vi "test progress notifications.vi"(8 "error in (no error)":errorcluster) -> (0 "error out":errorcluster, 3 "body":string)   [LabVIEW 2020, in "MCP Server tests.lvlib"]
doc: "Progress notifications over Server-Sent Events. fake_tool_progress works through 10 steps and calls Report Progress.vi before each. A tools/call with params._meta.progressToken whose Accept header contains text/event-stream is answered as text/event-stream: ten notifications/progress events carrying the progressToken exactly as sent (a string in the legacy request, a number in the modern one) with progress 1..10 in increasing order and total 10, then the JSON-RPC result as the last data event. The same call without a progressToken is answered as plain application/json. The requests are sent with the LabVIEW HTTP Client directly."
uses:
  MCP Server tests.lvlib
  <vilib>/addons/_JKI Toolkits/Caraya/classes/Test/Test.lvclass
  <vilib>/addons/_JKI Toolkits/Caraya/classes/Assert/Assert.lvclass
panel:
  out "lookup error":errorcluster
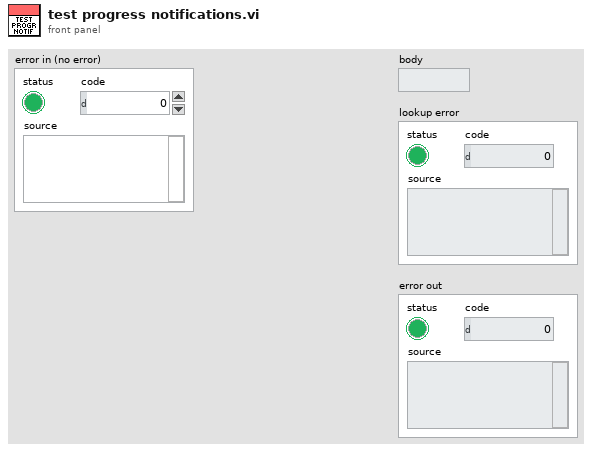
[diagram p1: front panel]
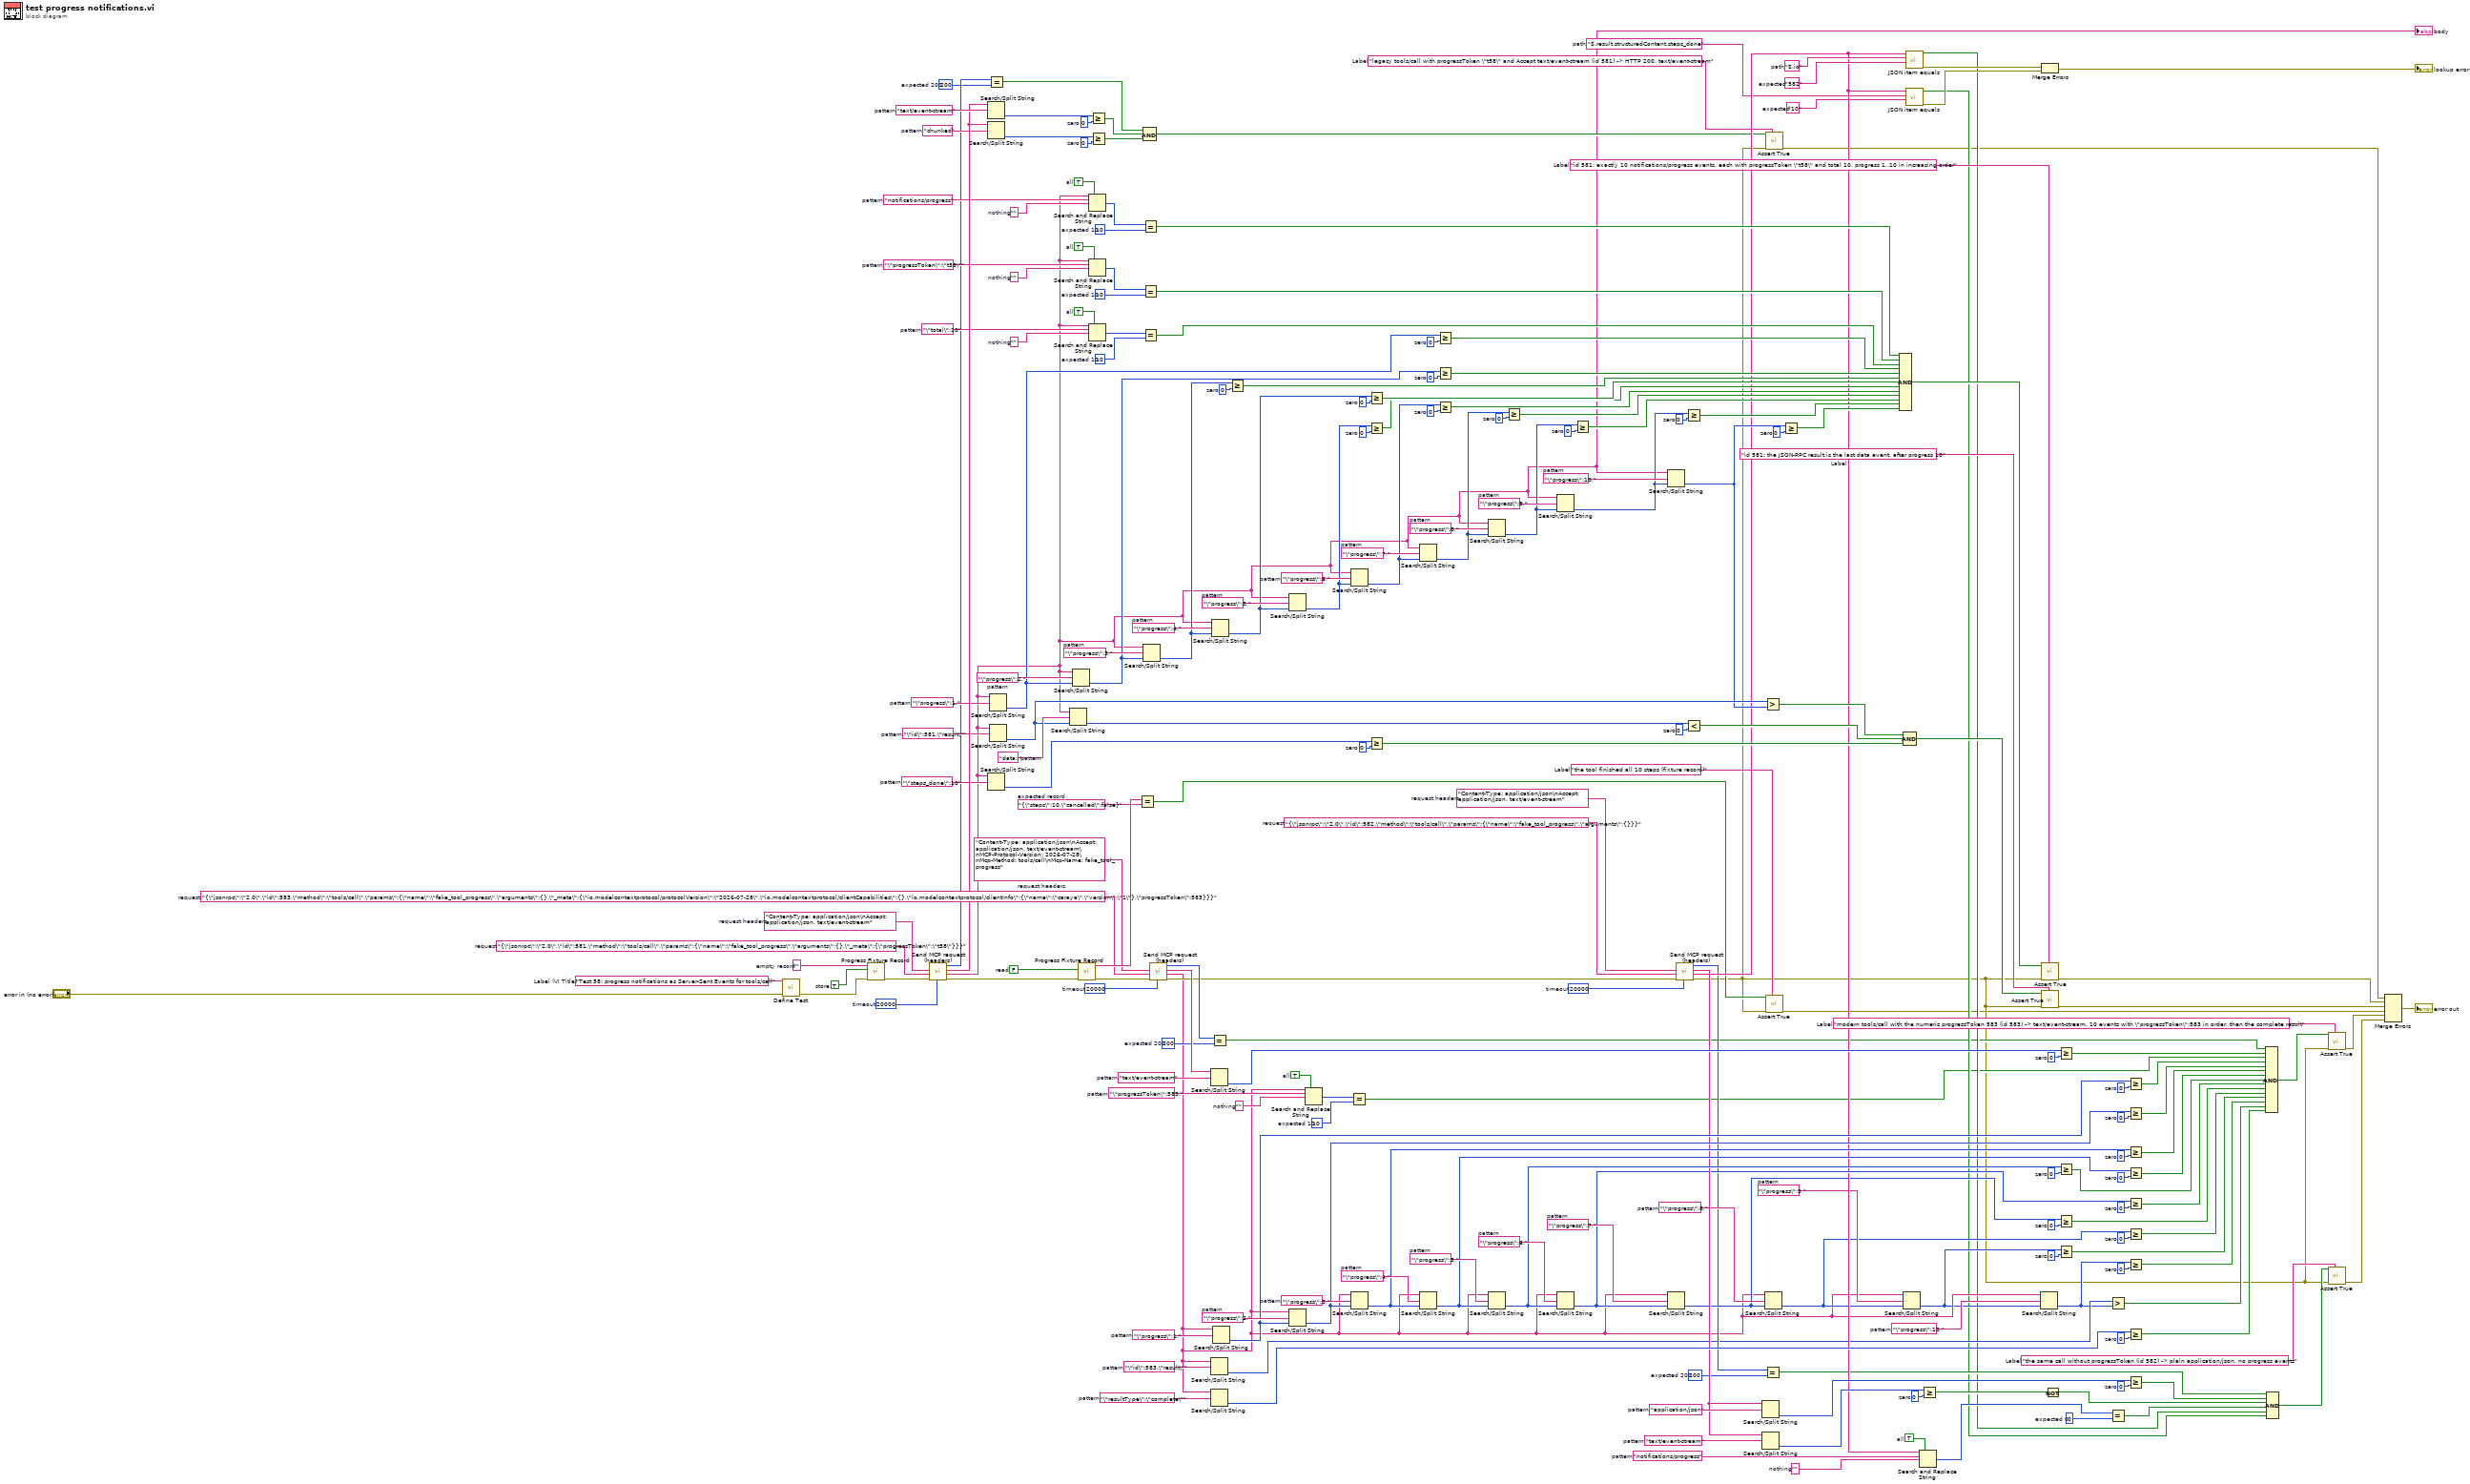
[diagram p0: block diagram]
diagram:
  w88 = "Content-Type: application/json\nAccept: application/json, text/event-stream"  # request headers
  w142 = "Content-Type: application/json\nAccept: application/json, text/event-stream\nMCP-Protocol-Version: 2026-07-28\nMcp-Method: tools/call\nMcp-Name: fake_tool_progress"  # request headers
  w209 = "Content-Type: application/json\nAccept: application/json, text/event-stream"  # request headers
  w28 = "the same call without progressToken (id 582) -> plain application/json, no progress events"  # Label
  w10 = "modern tools/call with the numeric progressToken 583 (id 583) -> text/event-stream, 10 events with \"progressToken\":583 in order, then the complete result"  # Label
  w52 = "the tool finished all 10 steps (fixture record)"  # Label
  w54 = "id 581: the JSON-RPC result is the last data event, after progress 10"  # Label
  w56 = "id 581: exactly 10 notifications/progress events, each with progressToken \"t58\" and total 10, progress 1..10 in increasing order"  # Label
  w58 = "legacy tools/call with progressToken \"t58\" and Accept text/event-stream (id 581) -> HTTP 200, text/event-stream"  # Label
  w61 = "10"  # expected
  w62 = "$.result.structuredContent.steps_done"  # path
  w65 = "582"  # expected
  w66 = "$.id"  # path
  w67 = 0  # expected 0
  w76 = TRUE  # all
  w77 = ""  # nothing
  w78 = "notifications/progress"  # pattern
  w69 = 0  # zero
  w79 = "text/event-stream"  # pattern
  w71 = 0  # zero
  w81 = "application/json"  # pattern
  w47 = 200  # expected 200
  w116 = 0  # zero
  w128 = "\"resultType\":\"complete\""  # pattern
  w129 = "\"id\":583,\"result\""  # pattern
  w118 = 10  # expected 10
  w130 = TRUE  # all
  w131 = ""  # nothing
  w132 = "\"progressToken\":583,"  # pattern
  w123 = 0  # zero
  w134 = "text/event-stream"  # pattern
  w114 = 200  # expected 200
  w38 = 0  # zero
  w40 = "\"progress\":10,"  # pattern
  w42 = 0  # zero
  w44 = "\"progress\":9,"  # pattern
  w45 = 0  # zero
  w50 = "\"progress\":8,"  # pattern
  w51 = 0  # zero
  w74 = "\"progress\":7,"  # pattern
  w75 = 0  # zero
  w83 = "\"progress\":6,"  # pattern
  w84 = 0  # zero
  w90 = "\"progress\":5,"  # pattern
  w91 = 0  # zero
  w93 = "\"progress\":4,"  # pattern
  w94 = 0  # zero
  w112 = "\"progress\":3,"  # pattern
  w113 = 0  # zero
  w121 = "\"progress\":2,"  # pattern
  w122 = 0  # zero
  w133 = "\"progress\":1,"  # pattern
  w164 = "{\"steps\":10,\"cancelled\":false}"  # expected record
  w175 = 0  # zero
  w191 = "\"steps_done\":10"  # pattern
  w166 = 0  # zero
  w183 = "data: "  # pattern
  w177 = 10  # expected 10
  w192 = TRUE  # all
  w193 = ""  # nothing
  w194 = "\"total\":10"  # pattern
  w179 = 10  # expected 10
  w195 = TRUE  # all
  w196 = ""  # nothing
  w197 = "\"progressToken\":\"t58\""  # pattern
  w181 = 10  # expected 10
  w198 = TRUE  # all
  w199 = ""  # nothing
  w200 = "notifications/progress"  # pattern
  w187 = 0  # zero
  w203 = "chunked"  # pattern
  w189 = 0  # zero
  w205 = "text/event-stream"  # pattern
  w171 = 200  # expected 200
  w201 = "\"id\":581,\"result\""  # pattern
  w127 = 0  # zero
  w137 = "\"progress\":10,"  # pattern
  w138 = 0  # zero
  w144 = "\"progress\":9,"  # pattern
  w145 = 0  # zero
  w147 = "\"progress\":8,"  # pattern
  w148 = 0  # zero
  w150 = "\"progress\":7,"  # pattern
  w151 = 0  # zero
  w153 = "\"progress\":6,"  # pattern
  w154 = 0  # zero
  w156 = "\"progress\":5,"  # pattern
  w157 = 0  # zero
  w162 = "\"progress\":4,"  # pattern
  w163 = 0  # zero
  w169 = "\"progress\":3,"  # pattern
  w170 = 0  # zero
  w185 = "\"progress\":2,"  # pattern
  w186 = 0  # zero
  w202 = "\"progress\":1,"  # pattern
  w86 = 20000  # timeout
  w87 = "{\"jsonrpc\":\"2.0\",\"id\":582,\"method\":\"tools/call\",\"params\":{\"name\":\"fake_tool_progress\",\"arguments\":{}}}"  # request
  w140 = 20000  # timeout
  w141 = "{\"jsonrpc\":\"2.0\",\"id\":583,\"method\":\"tools/call\",\"params\":{\"name\":\"fake_tool_progress\",\"arguments\":{},\"_meta\":{\"io.modelcontextprotocol/protocolVersion\":\"2026-07-28\",\"io.modelcontextprotocol/clientCapabilities\":{},\"io.modelcontextprotocol/clientInfo\":{\"name\":\"caraya\",\"version\":\"1\"},\"progressToken\":583}}}"  # request
  w174 = FALSE  # read
  w207 = 20000  # timeout
  w208 = "{\"jsonrpc\":\"2.0\",\"id\":581,\"method\":\"tools/call\",\"params\":{\"name\":\"fake_tool_progress\",\"arguments\":{},\"_meta\":{\"progressToken\":\"t58\"}}}"  # request
  w211 = TRUE  # store
  w212 = ""  # empty record
  w214 = "Test 58: progress notifications as Server-Sent Events for tools/call"  # Label (VI Title)
  n1 = call <vilib>:"Define Test.vi"("error in (no error)"="error in (no error)", "Label (VI Title)"=w214) -> ("error out"=w210:errorcluster)  [unwired: 8 in, 1 out]
  n2 = call "Progress Fixture Record.vi"("error in"=w210, "set?"=w211, "record in"=w212) -> ("error out"=w206:errorcluster)  [unwired: 7 in, 1 out]
  n3 = call "Send MCP request (headers).vi"("timeout (10000)"=w207, "error in (no error)"=w206, "request"=w208, "request headers"=w209) -> ("error out"=w173:errorcluster, "response"=w3:string, "headers"=w204:string, "status code"=w172:i32)  [unwired: 4 in]
  "body" <- w3
  n4 = Search/Split String(string=w204, search string/char (-)=w205) -> (offset of match=w190:i32)  [unwired: 1 in, 2 out]
  n5 = Search/Split String(string=w204, search string/char (-)=w203) -> (offset of match=w188:i32)  [unwired: 1 in, 2 out]
  n6 = Search/Split String(string=w3, search string/char (-)=w191) -> (offset of match=w176:i32)  [unwired: 1 in, 2 out]
  n7 = Equal?(x=w172, y=w171) -> (x = y?=w160:bool)
  n8 = Search/Split String(string=w3, search string/char (-)=w202) -> (offset of match=w184:i32)  [unwired: 1 in, 2 out]
  n9 = Search/Split String(string=w3, search string/char (-)=w201) -> (offset of match=w126:i32)  [unwired: 1 in, 2 out]
  n10 = Search/Split String(string=w3, search string/char (-)=w183, offset (0)=w126) -> (offset of match=w167:i32)  [unwired: 2 out]
  n11 = Search/Split String(string=w3, search string/char (-)=w185, offset (0)=w184) -> (offset of match=w168:i32)  [unwired: 2 out]
  n12 = call "Progress Fixture Record.vi"("error in"=w173, "set?"=w174) -> ("error out"=w139:errorcluster, "record out"=w165:string)  [unwired: 8 in]
  n13 = Search and Replace String(replace all?=w198, input string=w3, search string=w200, replace string=w199) -> (number of replacements=w182:i32)  [unwired: 4 in, 3 out]
  n14 = Search and Replace String(replace all?=w195, input string=w3, search string=w197, replace string=w196) -> (number of replacements=w180:i32)  [unwired: 4 in, 3 out]
  n15 = Search and Replace String(replace all?=w192, input string=w3, search string=w194, replace string=w193) -> (number of replacements=w178:i32)  [unwired: 4 in, 3 out]
  n16 = Greater Or Equal?(x=w190, y=w189) -> (x >= y?=w159:bool)
  n17 = Greater Or Equal?(x=w188, y=w187) -> (x >= y?=w158:bool)
  n18 = Equal?(x=w165, y=w164) -> (x = y?=w53:bool)
  n19 = Equal?(x=w182, y=w181) -> (x = y?=w110:bool)
  n20 = Equal?(x=w180, y=w179) -> (x = y?=w109:bool)
  n21 = Equal?(x=w178, y=w177) -> (x = y?=w108:bool)
  n22 = Search/Split String(string=w3, search string/char (-)=w169, offset (0)=w168) -> (offset of match=w161:i32)  [unwired: 2 out]
  n23 = Compound Arithmetic op=AND(w160, w159, w158) -> (w59:bool)
  n24 = call "Send MCP request (headers).vi"("timeout (10000)"=w140, "error in (no error)"=w139, "request"=w141, "request headers"=w142) -> ("error out"=w85:errorcluster, "response"=w41:string, "headers"=w135:string, "status code"=w115:i32)  [unwired: 4 in]
  n25 = Search/Split String(string=w135, search string/char (-)=w134) -> (offset of match=w124:i32)  [unwired: 1 in, 2 out]
  n26 = Search/Split String(string=w41, search string/char (-)=w129) -> (offset of match=w37:i32)  [unwired: 1 in, 2 out]
  n27 = Search/Split String(string=w41, search string/char (-)=w128) -> (offset of match=w117:i32)  [unwired: 1 in, 2 out]
  n28 = Equal?(x=w115, y=w114) -> (x = y?=w27:bool)
  n29 = Search/Split String(string=w3, search string/char (-)=w162, offset (0)=w161) -> (offset of match=w155:i32)  [unwired: 2 out]
  n30 = Search/Split String(string=w41, search string/char (-)=w133) -> (offset of match=w120:i32)  [unwired: 1 in, 2 out]
  n31 = Greater Or Equal?(x=w161, y=w163) -> (x >= y?=w105:bool)
  n32 = Search/Split String(string=w3, search string/char (-)=w156, offset (0)=w155) -> (offset of match=w152:i32)  [unwired: 2 out]
  n33 = Search/Split String(string=w41, search string/char (-)=w121, offset (0)=w120) -> (offset of match=w111:i32)  [unwired: 2 out]
  n34 = Search and Replace String(replace all?=w130, input string=w41, search string=w132, replace string=w131) -> (number of replacements=w119:i32)  [unwired: 4 in, 3 out]
  n35 = Equal?(x=w119, y=w118) -> (x = y?=w25:bool)
  n36 = Search/Split String(string=w3, search string/char (-)=w153, offset (0)=w152) -> (offset of match=w149:i32)  [unwired: 2 out]
  n37 = Search/Split String(string=w41, search string/char (-)=w112, offset (0)=w111) -> (offset of match=w92:i32)  [unwired: 2 out]
  n38 = Greater Or Equal?(x=w155, y=w157) -> (x >= y?=w104:bool)
  n39 = Greater Or Equal?(x=w152, y=w154) -> (x >= y?=w103:bool)
  n40 = Greater Or Equal?(x=w176, y=w175) -> (x >= y?=w95:bool)
  n41 = Search/Split String(string=w3, search string/char (-)=w150, offset (0)=w149) -> (offset of match=w146:i32)  [unwired: 2 out]
  n42 = Search/Split String(string=w41, search string/char (-)=w93, offset (0)=w92) -> (offset of match=w89:i32)  [unwired: 2 out]
  n43 = Greater Or Equal?(x=w184, y=w186) -> (x >= y?=w107:bool)
  n44 = Greater Or Equal?(x=w168, y=w170) -> (x >= y?=w106:bool)
  n45 = Greater Or Equal?(x=w149, y=w151) -> (x >= y?=w102:bool)
  n46 = Search/Split String(string=w3, search string/char (-)=w147, offset (0)=w146) -> (offset of match=w143:i32)  [unwired: 2 out]
  n47 = Search/Split String(string=w41, search string/char (-)=w90, offset (0)=w89) -> (offset of match=w82:i32)  [unwired: 2 out]
  n48 = Greater Or Equal?(x=w146, y=w148) -> (x >= y?=w101:bool)
  n49 = Search/Split String(string=w3, search string/char (-)=w144, offset (0)=w143) -> (offset of match=w136:i32)  [unwired: 2 out]
  n50 = Search/Split String(string=w41, search string/char (-)=w83, offset (0)=w82) -> (offset of match=w73:i32)  [unwired: 2 out]
  n51 = Greater Or Equal?(x=w143, y=w145) -> (x >= y?=w100:bool)
  n52 = Search/Split String(string=w3, search string/char (-)=w137, offset (0)=w136) -> (offset of match=w125:i32)  [unwired: 2 out]
  n53 = Search/Split String(string=w41, search string/char (-)=w74, offset (0)=w73) -> (offset of match=w49:i32)  [unwired: 2 out]
  n54 = call "Send MCP request (headers).vi"("timeout (10000)"=w86, "error in (no error)"=w85, "request"=w87, "request headers"=w88) -> ("error out"=w11:errorcluster, "response"=w63:string, "headers"=w80:string, "status code"=w48:i32)  [unwired: 4 in]
  n55 = Greater Or Equal?(x=w136, y=w138) -> (x >= y?=w99:bool)
  n56 = Less?(x=w167, y=w166) -> (x < y?=w96:bool)
  n57 = Search/Split String(string=w80, search string/char (-)=w81) -> (offset of match=w72:i32)  [unwired: 1 in, 2 out]
  n58 = Search/Split String(string=w80, search string/char (-)=w79) -> (offset of match=w70:i32)  [unwired: 1 in, 2 out]
  n59 = Greater?(x=w126, y=w125) -> (0:w97:bool)
  n60 = Search/Split String(string=w41, search string/char (-)=w50, offset (0)=w49) -> (offset of match=w43:i32)  [unwired: 2 out]
  n61 = Equal?(x=w48, y=w47) -> (x = y?=w35:bool)
  n62 = call <vilib>:"Assert True.vi"("Label"=w58, "error in (no error)"=w11, "True?"=w59) -> ("error out"=w9:errorcluster)  [unwired: 7 in, 1 out]
  n63 = call <vilib>:"Assert True.vi"("Label"=w52, "error in (no error)"=w11, "True?"=w53) -> ("error out"=w6:errorcluster)  [unwired: 7 in, 1 out]
  n64 = Greater Or Equal?(x=w125, y=w127) -> (x >= y?=w98:bool)
  n65 = Compound Arithmetic op=AND(w110, w109, w108, w107, w106, w105, w104, w103, w102, w101, w100, w99, w98) -> (w57:bool)
  n66 = Compound Arithmetic op=AND(w97, w96, w95) -> (w55:bool)
  n67 = Search/Split String(string=w41, search string/char (-)=w44, offset (0)=w43) -> (offset of match=w39:i32)  [unwired: 2 out]
  n68 = call "JSON item equals.vi"("expected"=w65, "path"=w66, "JSON"=w63) -> ("error out"=w64:errorcluster, "equal?"=w31:bool)  [unwired: 6 in, 1 out]
  n69 = call "JSON item equals.vi"("expected"=w61, "path"=w62, "JSON"=w63) -> ("error out"=w60:errorcluster, "equal?"=w30:bool)  [unwired: 6 in, 1 out]
  n70 = Search and Replace String(replace all?=w76, input string=w63, search string=w78, replace string=w77) -> (number of replacements=w68:i32)  [unwired: 4 in, 3 out]
  n71 = Greater Or Equal?(x=w70, y=w69) -> (x >= y?=w46:bool)
  n72 = Search/Split String(string=w41, search string/char (-)=w40, offset (0)=w39) -> (offset of match=w36:i32)  [unwired: 2 out]
  n73 = Merge Errors(w64, w60) -> (→"lookup error":errorcluster)
  n74 = call <vilib>:"Assert True.vi"("Label"=w56, "error in (no error)"=w11, "True?"=w57) -> ("error out"=w8:errorcluster)  [unwired: 7 in, 1 out]
  n75 = call <vilib>:"Assert True.vi"("Label"=w54, "error in (no error)"=w11, "True?"=w55) -> ("error out"=w7:errorcluster)  [unwired: 7 in, 1 out]
  n76 = Not(x=w46) -> (.not. x?=w33:bool)
  n77 = Greater Or Equal?(x=w124, y=w123) -> (x >= y?=w26:bool)
  n78 = Greater Or Equal?(x=w82, y=w84) -> (x >= y?=w20:bool)
  n79 = Greater Or Equal?(x=w49, y=w51) -> (x >= y?=w18:bool)
  n80 = Greater Or Equal?(x=w39, y=w42) -> (x >= y?=w16:bool)
  n81 = Greater?(x=w37, y=w36) -> (0:w14:bool)
  n82 = Equal?(x=w68, y=w67) -> (x = y?=w32:bool)
  n83 = Greater Or Equal?(x=w120, y=w122) -> (x >= y?=w24:bool)
  n84 = Greater Or Equal?(x=w111, y=w113) -> (x >= y?=w23:bool)
  n85 = Greater Or Equal?(x=w92, y=w94) -> (x >= y?=w22:bool)
  n86 = Greater Or Equal?(x=w89, y=w91) -> (x >= y?=w21:bool)
  n87 = Greater Or Equal?(x=w73, y=w75) -> (x >= y?=w19:bool)
  n88 = Greater Or Equal?(x=w43, y=w45) -> (x >= y?=w17:bool)
  n89 = Greater Or Equal?(x=w36, y=w38) -> (x >= y?=w15:bool)
  n90 = Greater Or Equal?(x=w117, y=w116) -> (x >= y?=w13:bool)
  n91 = Greater Or Equal?(x=w72, y=w71) -> (x >= y?=w34:bool)
  n92 = Compound Arithmetic op=AND(w27, w26, w25, w24, w23, w22, w21, w20, w19, w18, w17, w16, w15, w14, w13) -> (w12:bool)
  n93 = Compound Arithmetic op=AND(w35, w34, w33, w32, w31, w30) -> (w29:bool)
  n94 = call <vilib>:"Assert True.vi"("Label"=w10, "error in (no error)"=w11, "True?"=w12) -> ("error out"=w5:errorcluster)  [unwired: 7 in, 1 out]
  n95 = call <vilib>:"Assert True.vi"("Label"=w28, "error in (no error)"=w11, "True?"=w29) -> ("error out"=w4:errorcluster)  [unwired: 7 in, 1 out]
  n96 = Merge Errors(w9, w8, w7, w6, w5, w4) -> (→"error out":errorcluster)
